vi "RDC-test-check_perm.vi"() -> ()   [LabVIEW 2020]
doc: "Test panel, run by hand: compares calculated permittivity and impedance with reference data on tabs Compare, Impedance and Error Check. It reads common-format files and uses the linear correction VIs and the water model."
uses:
  RDC-error_metric_clust.ctl
  Reflector/RFH-common_data_format.ctl
  RDC-Reflection_Data_Computation.lvlib
  Reflector/RFH-Reflection_File_Handler.lvlib
panel:
  out "element 2":string
  in  "water Temp (25C) [10-40C]  2":dbl=22.5
  in  "comp data":i32=3
  in  "stop":bool
  out "element":string
  in  "Tab Control":enum32{"Compare", "Impedance", "Error Check"}(tab)
  out "Real Perm":T1(graph)
  out "Tau":dbl format="%#_6p"
  out "C0":dbl format="%#_6p"
  out "Imag Perm":T1(graph)
  out "C0 2":dbl format="%#_6p"
  in  "C0 set":dbl format="%#_6p"
  out "Reactance":cluster{"Frequency":dbl[], dbl[]}[](graph)
  out "Resistance":cluster{"Frequency":dbl[], dbl[]}[](graph)
  out "Smith Plot":picture
  out "Diff Real":dbl[](graph)
  out "Diff Imag":dbl[](graph)
  out "percent diff real":dbl[](graph)
  out "percent diff imag":dbl[](graph)
  out "Error Metric":T2
  in  "data":i32=3
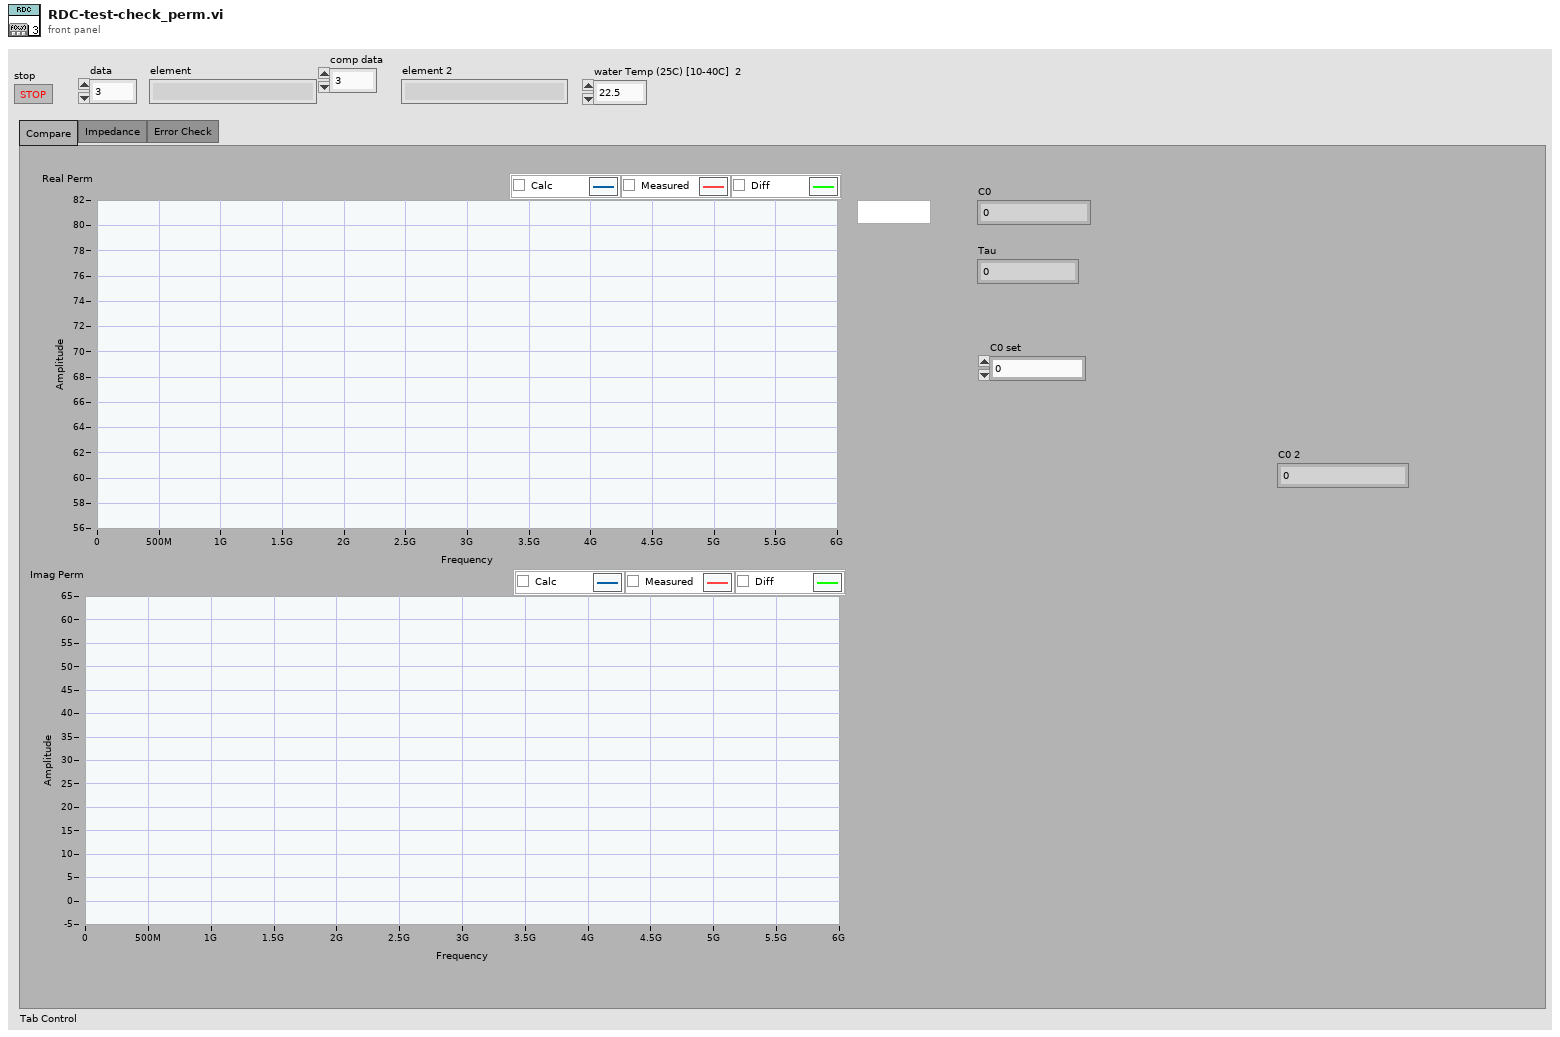
[diagram p1: front panel]
types:
  T1 = cluster{"Frequency":dbl[], "Permativity'":dbl[]}[]
  T2 = typedef "RDC-Reflection_Data_Computation.lvlib/RDC-error_metric_clust.ctl" = cluster{"Diff":cdb[], "percent diff":cdb[], "Average diff":cdb, "Percent avg diff":cdb, "RMSE diff":cdb}
  T3 = typedef "RFH-Reflection_File_Handler.lvlib/RFH-common_data_format.ctl" = cluster{"Frequency":dbl[], "Reflection'":dbl[], "Reflection''":dbl[], "Permativity'":dbl[], "Permativity''":dbl[], "Conductivity":dbl[], "Loss Tangent":dbl[], "Resistance":dbl[], "Reactance":dbl[]}
  T4 = cluster{"left":i16, "top":i16, "right":i16, "bottom":i16}
  T5 = cluster{"x minimum":dbl, "x maximum":dbl, "y minimum":dbl, "y maximum":dbl}
  T6 = cluster{"normalized smith points {r,x}":cluster{"r":dbl, "x":dbl}[]}[]
  T7 = cluster{"Frequency":dbl[], "Permativity''":dbl[]}
  T8 = cluster{"Frequency":dbl[], "Permativity''":dbl[]}[]
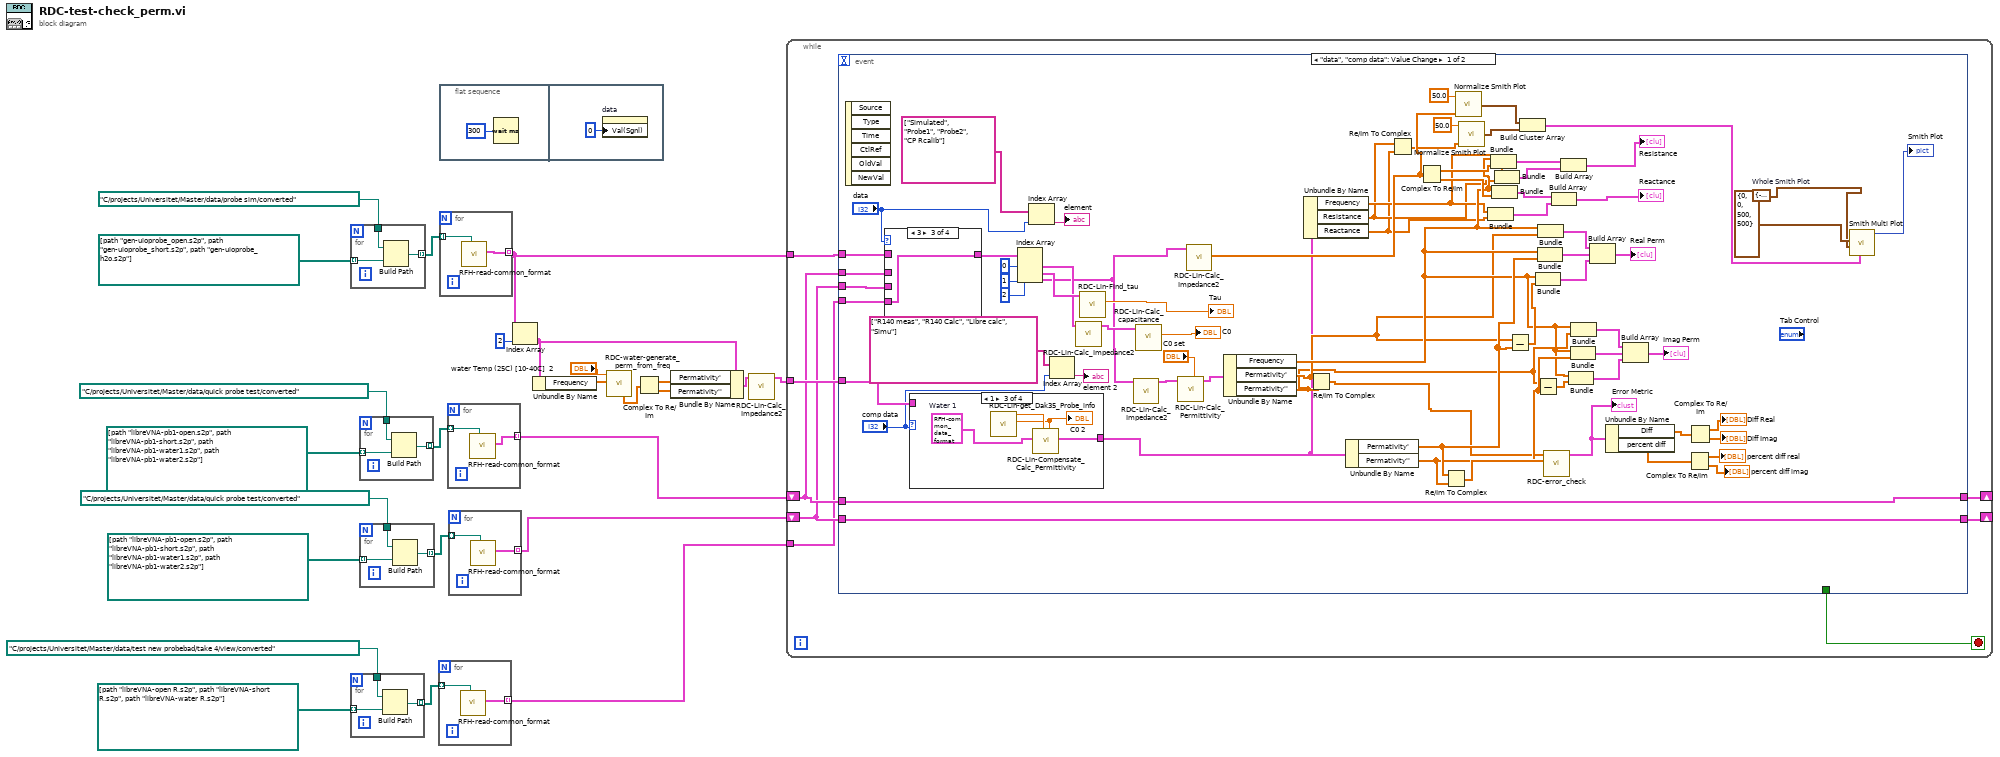
[diagram p0: block diagram]
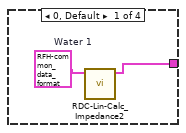
[diagram p5: hidden frame]
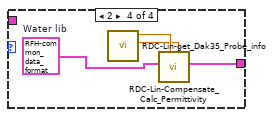
[diagram p7: hidden frame]
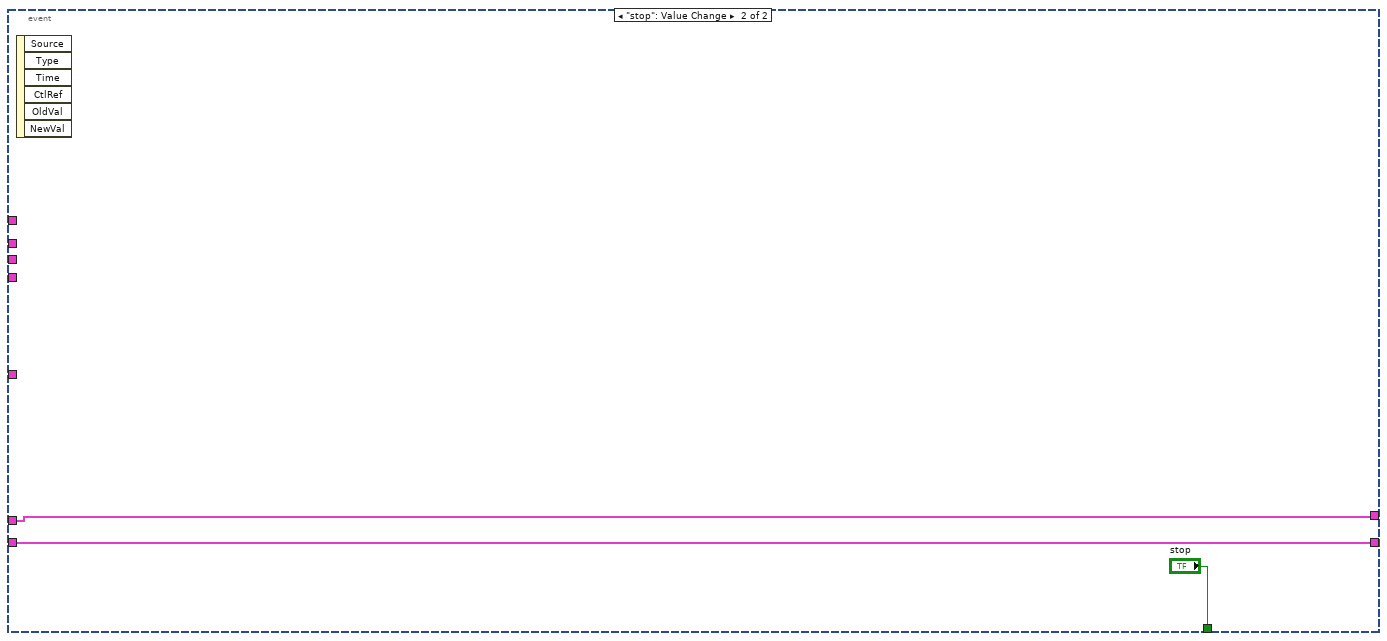
[diagram p8: hidden frame]
diagram:
  n1 = for {
    tunnel: path "C:/projects/Universitet/Master/data/test new probebad/take 4/view/converted" ("base path") -> [w28]
    tunnel: [w27] -> w3 mode=indexing
    tunnel: path[] [path "libreVNA-open R.s2p", path "libreVNA-short R.s2p", path "libreVNA-water R.s2p"] ("file path (dialog if empty)") -> [w26] mode=indexing
    n2 = Build Path(base path=w28, name or relative path=w26) -> (appended path=w27:path)
  }
  n3 = for {
    tunnel: path "C:/projects/Universitet/Master/data/probe sim/converted" ("base path") -> [w31]
    tunnel: [w30] -> w24 mode=indexing
    tunnel: path[] [path "gen-uioprobe_open.s2p", path "gen-uioprobe_short.s2p", path "gen-uioprobe_h2o.s2p"] ("file path (dialog if empty)") -> [w29] mode=indexing
    n4 = Build Path(base path=w31, name or relative path=w29) -> (appended path=w30:path)
  }
  n5 = for {
    tunnel: path "C:/projects/Universitet/Master/data/quick probe test/converted" ("base path") -> [w34]
    tunnel: [w33] -> w21 mode=indexing
    tunnel: path[] [path "libreVNA-pb1-open.s2p", path "libreVNA-pb1-short.s2p", path "libreVNA-pb1-water1.s2p", path "libreVNA-pb1-water2.s2p"] ("file path (dialog if empty)") -> [w32] mode=indexing
    n6 = Build Path(base path=w34, name or relative path=w32) -> (appended path=w33:path)
  }
  n7 = for {
    tunnel: path "C:/projects/Universitet/Master/data/quick probe test/converted" ("base path") -> [w37]
    tunnel: [w36] -> w18 mode=indexing
    tunnel: path[] [path "libreVNA-pb1-open.s2p", path "libreVNA-pb1-short.s2p", path "libreVNA-pb1-water1.s2p", path "libreVNA-pb1-water2.s2p"] ("file path (dialog if empty)") -> [w35] mode=indexing
    n8 = Build Path(base path=w37, name or relative path=w35) -> (appended path=w36:path)
  }
  n9 = for {
    tunnel: w3 -> [w39] mode=indexing
    tunnel: [w38] -> w1 mode=indexing
    n10 = call "RFH-read-common_format.vi"("file path (dialog if empty)"=w39) -> ("Common Format"=w38:T3)  [unwired: 9 in, 1 out]
  }
  n11 = flat-sequence {
    frame #0 {
      n12 = Wait (ms)(milliseconds to wait=u32 300) -> ()  [unwired: 1 out]
    }
    frame #1 {
      n13 = property on="data" class="DigNum (strict)"("Val(Sgnl)"=0 ("Value (Signaling)")) -> ()  [unwired: 2 in, 2 out]
    }
  }
  n14 = for {
    tunnel: w24 -> [w43] mode=indexing
    tunnel: [w42] -> w7 mode=indexing
    n15 = call "RFH-read-common_format.vi"("file path (dialog if empty)"=w43) -> ("Common Format"=w42:T3)  [unwired: 9 in, 1 out]
  }
  n16 = for {
    tunnel: w21 -> [w45] mode=indexing
    tunnel: [w44] -> w9 mode=indexing
    n17 = call "RFH-read-common_format.vi"("file path (dialog if empty)"=w45) -> ("Common Format"=w44:T3)  [unwired: 9 in, 1 out]
  }
  n18 = for {
    tunnel: w18 -> [w47] mode=indexing
    tunnel: [w46] -> w8 mode=indexing
    n19 = call "RFH-read-common_format.vi"("file path (dialog if empty)"=w47) -> ("Common Format"=w46:T3)  [unwired: 9 in, 1 out]
  }
  n20 = Index Array(array=w7, index=2) -> (element=w13:T3)
  n21 = Unbundle By Name(w13) -> ("Frequency"=w15:dbl[])
  n22 = call "RDC-water-generate_perm_from_freq.vi"("Frequency"=w15, "water Temp (25C) [10-40C]"="water Temp (25C) [10-40C]  2") -> ("Complex perm"=w12:cdb[])  [unwired: 5 in, 4 out]
  n23 = Complex To Re/Im(x + iy=w12) -> (x=w11:dbl[], y=w10:dbl[])
  n24 = Bundle By Name(cluster=w13, "Permativity'"=w11, "Permativity''"=w10) -> (w6:T3)
  n25 = call "RDC-Lin-Calc_Impedance2.vi"("input cluster"=w6) -> ("Output cluster"=w5:T3)  [unwired: 9 in, 1 out]
  n26 = while {
    tunnel: w5 -> [w54]
    shift-right: [w52] -> _
    shift-left: w9 -> [w51]
    shift-right: [w50] -> _
    shift-left: w8 -> [w49]
    tunnel: w7 -> [w53]
    tunnel: w1 -> [w48]
    stop <- w55 stop-if-true
    n27 = event shown="[0] \"data\", \"comp data\": Value Change" {
      selector: _ -> [_ _]
      dyn-events: _ -> [_ _]
      timeout: _ -> [_ _]
      tunnel: [_ "stop"] -> w55
      tunnel: w54 -> [w97 _]
      tunnel: w53 -> [w96 _]
      tunnel: w51 -> [w95 _]
      tunnel: w49 -> [w94 _]
      tunnel: [w90 w144] -> w52
      tunnel: w51 -> [w90 w144]
      tunnel: [w89 w143] -> w50
      tunnel: w49 -> [w89 w143]
      tunnel: w48 -> [w57 _]
      event "data", "comp data": Value Change {
        w66 = T5 {"x minimum"=-1.0, "x maximum"=1.0, "y minimum"=-1.0, "y maximum"=1.0}  # Whole Smith Plot
        n28 = event-data() -> ()  [unwired: 1 in, 6 out]
        n29 = case shown="3" "data" {
          tunnel: w96 -> [w128 _ _ _]
          tunnel: w95 -> [_ w129 _ _]
          tunnel: w94 -> [_ _ _ w131]
          tunnel: [w128 w129 w130 w131] -> w92
          tunnel: w57 -> [_ _ w130 _]
          frame 0, Default {
          }
          frame 1 {
          }
          frame 3 {
          }
          frame 2 {
          }
        }
        n30 = case shown="1" "comp data" {
          tunnel: [w132 w134 w135 w140] -> w73
          tunnel: w97 -> [_ w134 _ _]
          frame 0, Default {
            w133 = T3 {"Frequency"=array[2001 elements], "Reflection'"=array[2001 elements], "Reflection''"=array[2001 elements], "Permativity'"=array[2001 elements], "Permativity''"=array[2001 elements], "Conductivity"=array[2001 elements], "Loss Tangent"=array[2001 elements], "Resistance"=[], "Reactance"=[]}  # Water 1
            n31 = call "RDC-Lin-Calc_Impedance2.vi"("input cluster"=w133) -> ("Output cluster"=w132:T3)  [unwired: 9 in, 1 out]
          }
          frame 3 {
          }
          frame 1 {
            w136 = T3 {"Frequency"=array[2001 elements], "Reflection'"=array[2001 elements], "Reflection''"=array[2001 elements], "Permativity'"=array[2001 elements], "Permativity''"=array[2001 elements], "Conductivity"=array[2001 elements], "Loss Tangent"=array[2001 elements], "Resistance"=[], "Reactance"=[]}  # Water 1
            n32 = call "RDC-Lin-get_Dak35_Probe_info.vi"() -> ("C0"=w137:dbl, "Tau"=w138:dbl)  [unwired: 10 in]
            "C0 2" <- w137
            n33 = call "RDC-Lin-Compensate_Calc_Permittivity.vi"("C0"=w137, "Tau"=w138, "input cluster"=w136) -> ("Output cluster"=w135:T3)  [unwired: 8 in]
          }
          frame 2 {
            w139 = T3 {"Frequency"=array[2001 elements], "Reflection'"=array[2001 elements], "Reflection''"=array[2001 elements], "Permativity'"=array[2001 elements], "Permativity''"=array[2001 elements], "Conductivity"=array[2001 elements], "Loss Tangent"=array[2001 elements], "Resistance"=[], "Reactance"=[]}  # Water lib
            n34 = call "RDC-Lin-get_Dak35_Probe_info.vi"() -> ("C0"=w141:dbl, "Tau"=w142:dbl)  [unwired: 10 in]
            n35 = call "RDC-Lin-Compensate_Calc_Permittivity.vi"("C0"=w141, "Tau"=w142, "input cluster"=w139) -> ("Output cluster"=w140:T3)  [unwired: 8 in]
          }
        }
        n36 = Index Array(array=w92, index #1=0 ("index"), index #2=1 ("index"), index #3=2 ("index")) -> (element #1=w80:T3, element #2=w86:T3, element #3=w75:T3)
        n37 = Index Array(array=string[] ["Simulated", "Probe1", "Probe2", "CP Rcalib"], index="data") -> (element=→"element":string)
        n38 = Index Array(array=string[] ["R140 meas", "R140 Calc", "Libre calc", "Simu"], index="comp data") -> (element=→"element 2":string)
        n39 = call "RDC-Lin-Calc_Impedance2.vi"("input cluster"=w80) -> ("Output cluster"=w79:T3)  [unwired: 9 in, 1 out]
        n40 = call "RDC-Lin-Find_tau.vi"("Short Probe reading"=w86) -> ("Tau"=→"Tau":dbl)  [unwired: 9 in, 1 out]
        n41 = call "RDC-Lin-Calc_Impedance2.vi"("input cluster"=w75) -> ("Output cluster"=w76:T3)  [unwired: 9 in, 1 out]
        n42 = call "RDC-Lin-Calc_capacitance.vi"("Open Probe reading"=w79) -> ("C0"=→"C0":dbl)  [unwired: 9 in, 1 out]
        n43 = call "RDC-Lin-Calc_Permittivity.vi"("C0"="C0 set", "input cluster"=w76) -> ("Output cluster"=w77:T3)  [unwired: 9 in]
        n44 = call "RDC-Lin-Calc_Impedance2.vi"("input cluster"=w75) -> ("Impedance"=w74:cdb[])  [unwired: 9 in, 1 out]
        n45 = Unbundle By Name(w77) -> ("Frequency"=w104:dbl[], "Permativity'"=w100:dbl[], "Permativity''"=w99:dbl[])
        n46 = Unbundle By Name(w73) -> ("Frequency"=w72:dbl[], "Resistance"=w63:dbl[], "Reactance"=w62:dbl[])
        n47 = Re/Im To Complex(1:w99, 2:w100) -> (0:w98:cdb[])
        n48 = Unbundle By Name(w73) -> ("Permativity'"=w118:dbl[], "Permativity''"=w107:dbl[])
        n49 = Re/Im To Complex(1:w62, 2:w63) -> (0:w61:cdb[])
        n50 = Complex To Re/Im(x + iy=w74) -> (x=w106:dbl[], y=w105:dbl[])
        n51 = Re/Im To Complex(1:w107, 2:w118) -> (0:w120:cdb[])
        n52 = call <vilib>:"Normalize Smith Plot.vi"("points complex"=w74, "Zo (50.0)"=50.0) -> ("normalized smith points {r,x}"=w59:cluster{"r":dbl, "x":dbl}[])  [unwired: 1 in]
        n53 = call <vilib>:"Normalize Smith Plot.vi"("points complex"=w61, "Zo (50.0)"=50.0) -> ("normalized smith points {r,x}"=w60:cluster{"r":dbl, "x":dbl}[])  [unwired: 1 in]
        n54 = Bundle("Frequency"=w72, "Reactance"=w62) -> (w70:cluster{"Frequency":dbl[], "Reactance":dbl[]})  [unwired: 1 in]
        n55 = Bundle("Frequency"=w104, w106) -> (w103:cluster{"Frequency":dbl[], dbl[]})  [unwired: 1 in]
        n56 = Bundle("Frequency"=w104, w105) -> (w102:cluster{"Frequency":dbl[], dbl[]})  [unwired: 1 in]
        n57 = Bundle("Frequency"=w72, "Resistance"=w63) -> (w68:cluster{"Frequency":dbl[], "Resistance":dbl[]})  [unwired: 1 in]
        n58 = Subtract(x=w100, y=w118) -> (x-y=w113:dbl[])
        n59 = Build Cluster Array(w59, w60) -> (w58:T6)
        n60 = Bundle("Frequency"=w104, w113) -> (w115:cluster{"Frequency":dbl[], dbl[]})  [unwired: 1 in]
        n61 = Subtract(x=w99, y=w107) -> (x-y=w108:dbl[])
        n62 = Bundle("Frequency"=w104, "Permativity'"=w118) -> (w116:cluster{"Frequency":dbl[], "Permativity'":dbl[]})  [unwired: 1 in]
        n63 = Bundle("Frequency"=w104, "Permativity'"=w100) -> (w117:cluster{"Frequency":dbl[], "Permativity'":dbl[]})  [unwired: 1 in]
        n64 = call "RDC-error_check.vi"("Reference"=w120, "Calculated"=w98) -> ("Error Metric"=w121:T2)  [unwired: 9 in]
        "Error Metric" <- w121
        n65 = Build Array(w102, w70) -> (→"Reactance":cluster{"Frequency":dbl[], "Reactance":dbl[]}[])
        n66 = Build Array(w103, w68) -> (→"Resistance":cluster{"Frequency":dbl[], "Resistance":dbl[]}[])
        n67 = Bundle("Frequency"=w104, w108) -> (w111:cluster{"Frequency":dbl[], dbl[]})  [unwired: 1 in]
        n68 = Bundle("Frequency"=w104, "Permativity''"=w107) -> (w110:T7)  [unwired: 1 in]
        n69 = Bundle("Frequency"=w104, "Permativity''"=w99) -> (w109:T7)  [unwired: 1 in]
        n70 = Build Array(w117, w116, w115) -> (→"Real Perm":T1)
        n71 = Unbundle By Name(w121) -> ("Diff"=w122:cdb[], "percent diff"=w123:cdb[])
        n72 = Build Array(w109, w110, w111) -> (→"Imag Perm":T8)
        n73 = Complex To Re/Im(x + iy=w123) -> (x=→"percent diff real":dbl[], y=→"percent diff imag":dbl[])
        n74 = Complex To Re/Im(x + iy=w122) -> (x=→"Diff Real":dbl[], y=→"Diff Imag":dbl[])
        n75 = call <vilib>:"Smith Multi Plot.vi"("smith multi plot"=w58, "smith plot section"=w66, "rect"=T4 {"left"=0, "top"=0, "right"=500, "bottom"=500}) -> ("new picture"=→"Smith Plot":picture)  [unwired: 8 in]
      }
      event "stop": Value Change {
        n76 = event-data() -> ()  [unwired: 1 in, 6 out]
      }
    }
  }
